vi "Load Config.vi"(8 "error in (no error)":errorcluster, 11 "Data Processor Module in":refnum<class "Data Processor Module.lvclass">) -> (0 "error out":errorcluster, 3 "Data Processor Module out":refnum<class "Data Processor Module.lvclass">)   [LabVIEW 2020, in "VolatusData.lvlib" / "Data Processor Module.lvclass"]
uses:
  Data Processor Module.lvclass
  C:/dev/lv20CE/relink/lv-volatus/Volatus/Module/Module.lvclass
  Volatus/Module/Module.lvclass/Module.ctl
  VolatusConfig/VolatusConfigElement/VolatusConfigElement.lvclass/VolatusConfigElement.ctl
  Data Processor Module.lvclass/Data Processor Module.ctl
  VolatusConfig/VolatusConfigElement/Element.vi
  Volatus/Module/Module.lvclass
  VolatusConfig/VolatusConfigElement/VolatusConfigElement.lvclass
  lv-cdm/CDM-Config/Config Element/Config Element.lvclass
  C:/dev/lv20CE/relink/lv-volatus/VolatusData/Data Processor Module/Data Processor Module.lvclass
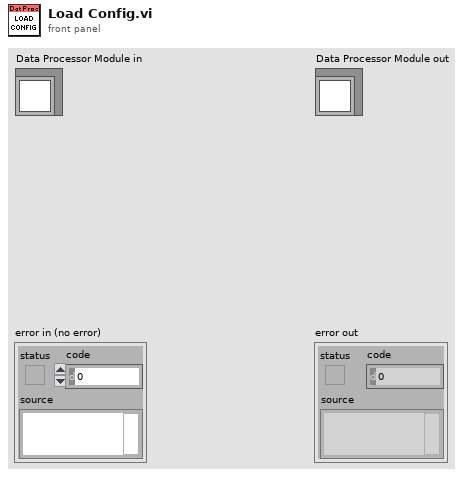
[diagram p1: front panel]
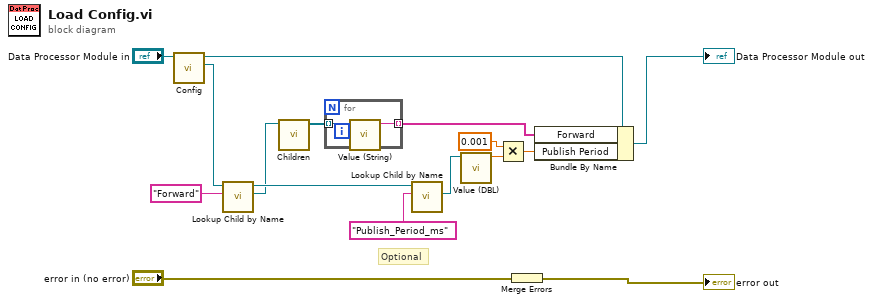
[diagram p0: block diagram]
diagram:
  # "Optional"
  n1 = call "Config.vi"("Module in"="Data Processor Module in") -> ("Config"=w6:refnum<class "VolatusConfigElement.lvclass">, "Module out"=w14:refnum<class "Data Processor Module.lvclass">)  [unwired: 9 in]
  n2 = call "Lookup Child by Name.vi"("Child Name"="Forward", "VolatusConfigElement in"=w6) -> ("Child"=w3:refnum<class "Config Element.lvclass">, "VolatusConfigElement out"=w5:refnum<class "VolatusConfigElement.lvclass">)  [unwired: 6 in, 2 out]
  n3 = call "Children.vi"("Config Element in"=w3) -> ("Elements"=w2:refnum<class "Config Element.lvclass">[])  [unwired: 9 in, 1 out]
  n4 = for {
    tunnel: w2 -> [w18] mode=indexing
    tunnel: [w17] -> w1 mode=indexing
    n5 = call "Value (String).vi"("Config Element in"=w18) -> ("String Value"=w17:string)  [unwired: 9 in, 1 out]
  }
  n6 = call "Lookup Child by Name.vi"("Child Name"="Publish_Period_ms", "VolatusConfigElement in"=w5) -> ("Child"=w12:refnum<class "Config Element.lvclass">)  [unwired: 6 in, 3 out]
  n7 = call "Value (DBL).vi"("Config Element in"=w12) -> ("DBL Value"=w11:dbl)  [unwired: 9 in, 1 out]
  n8 = Multiply(x=0.001, y=w11) -> (x*y=w8:dbl)
  n9 = Merge Errors("error in (no error)") -> (→"error out":errorcluster)
  n10 = Bundle By Name(cluster=w14, "Forward"=w1, "Publish Period"=w8) -> (→"Data Processor Module out":refnum<class "Data Processor Module.lvclass">)
